vi "FunctionGeneratorMatrix_Add_Value.vi"(9 "Y Value":T1, 10 "X Value":dbl, 11 "in FUNC_GEN_MATRIX":T2) -> (0 "Error":bool, 3 "out FUNC_GEN_MATRIX":T2)   [LabVIEW 2019, in "Trajectory_Library.lvlib"]
doc: "Insert new X, Y pair into an existing Function Generator Matrix data cluster.\n\nInputs:\n - Input Funct Gen Matrix -- Data cluster\n - X Value -- New X value\n - Y Value -- New Y matrix\n\nOutputs:\n - Function Generator Matrix -- Updated data cluster\n - Error -- Set true if an error occured. This is set when the size of the Y matrix does not match the definiton of this function generator."
uses:
  Trajectory_Library.lvlib
  TypeDef/FUNCTION_GENERATOR_MATRIX.ctl
  <vilib>/Analysis/Matrix/Datatypes/RealMatrix.ctl
  <vilib>/gmath/NI_Gmath.lvlib
  <vilib>/Analysis/Matrix/NI_Matrix.lvlib
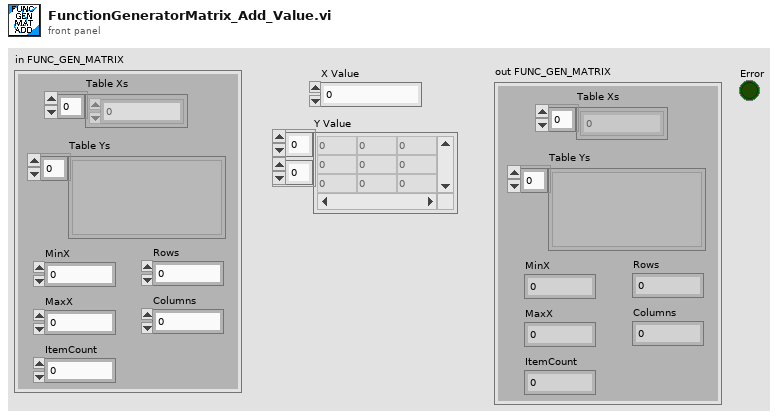
[diagram p1: front panel]
types:
  T1 = typedef "NI_Matrix.lvlib/RealMatrix.ctl" = dbl[][]
  T2 = typedef "Trajectory_Library.lvlib/FUNCTION_GENERATOR_MATRIX.ctl" = cluster{"Table Xs":dbl[], "Table Ys":variant[], "MinX":dbl, "MaxX":dbl, "ItemCount":i32, "Rows":i32, "Columns":i32}
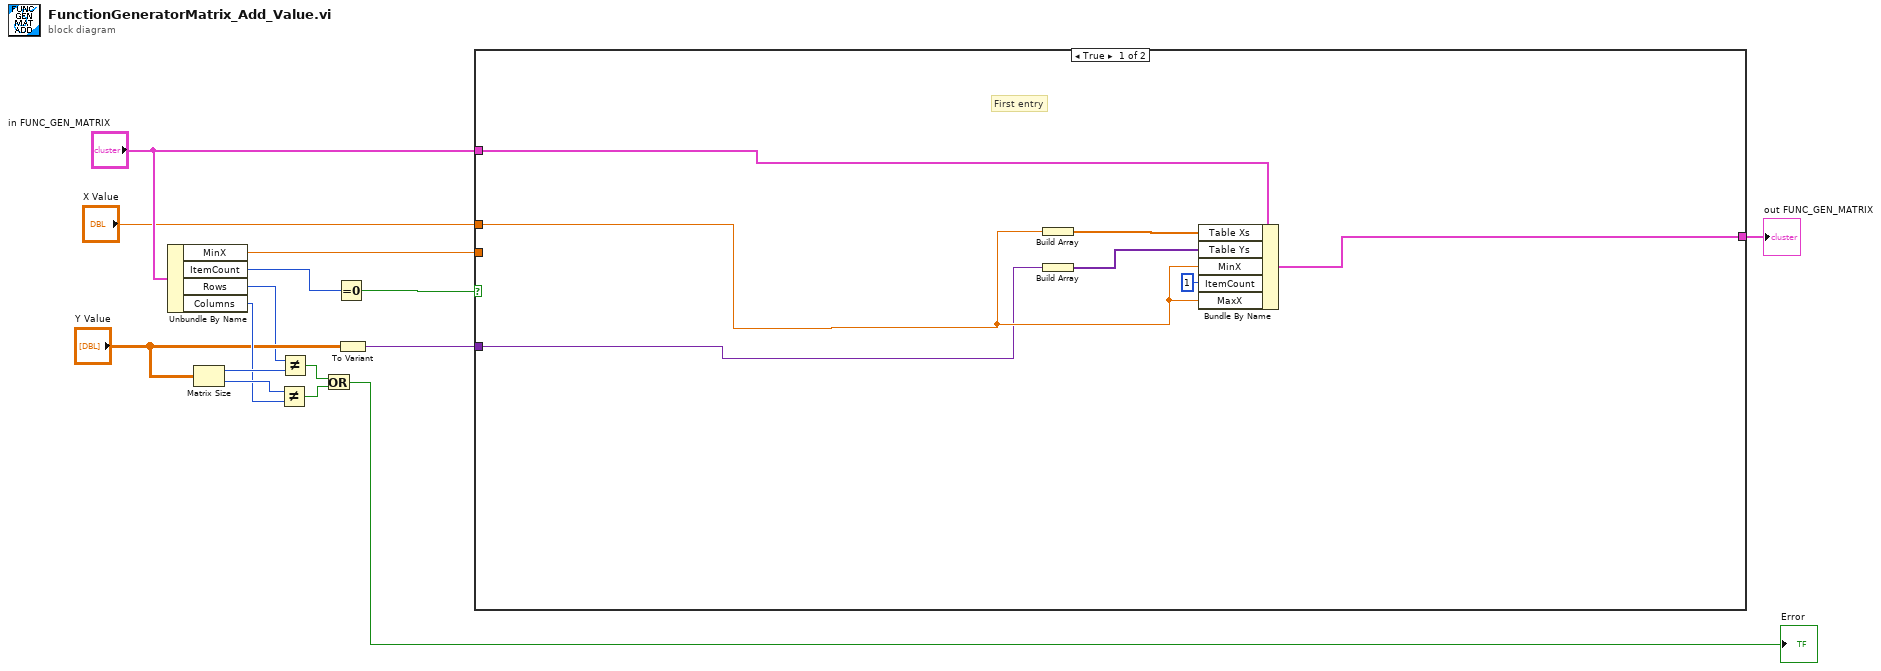
[diagram p0: block diagram]
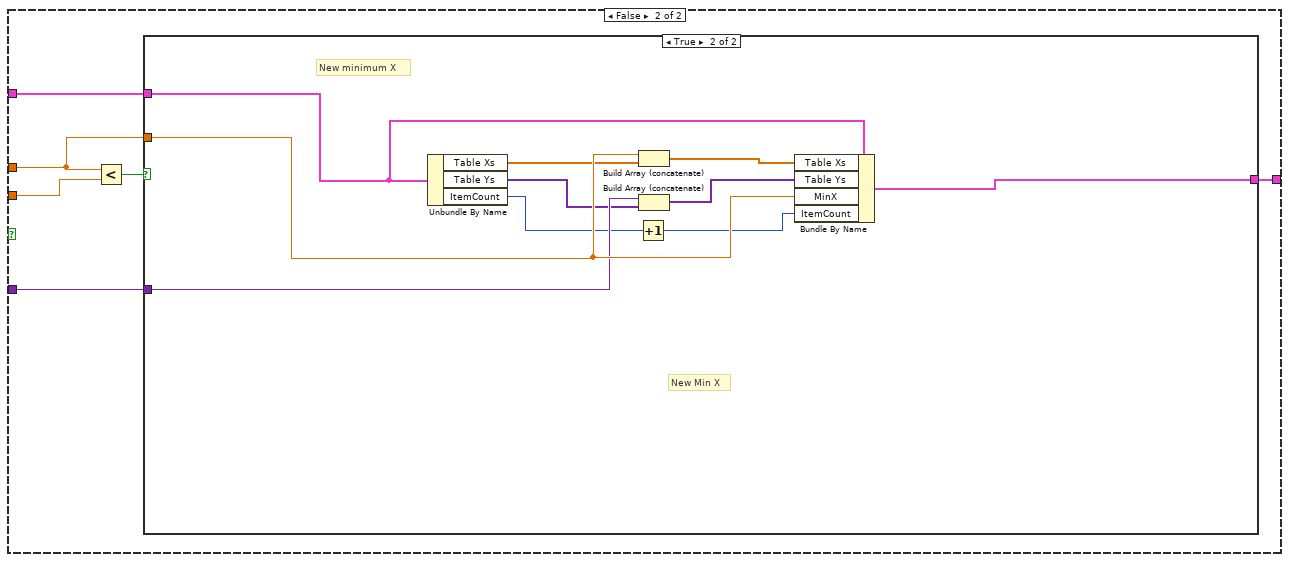
[diagram p2: hidden frame]
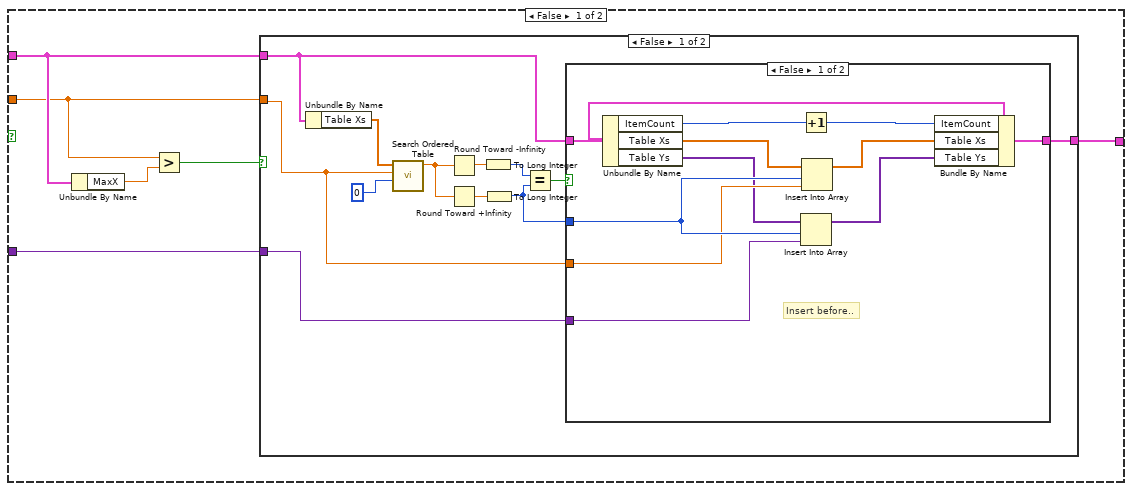
[diagram p3: hidden frame]
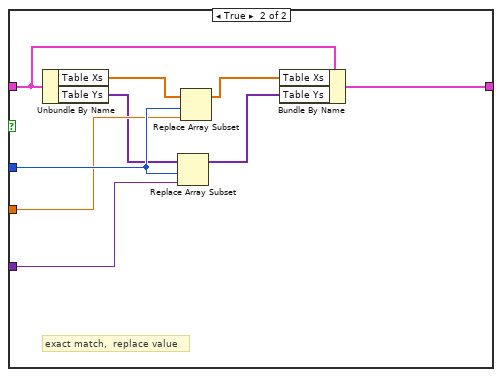
[diagram p4: hidden frame]
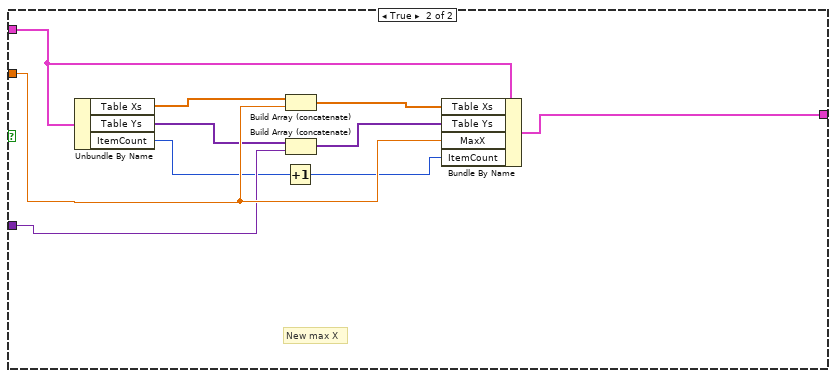
[diagram p5: hidden frame]
diagram:
  n1 = Unbundle By Name("in FUNC_GEN_MATRIX") -> ("MinX"=w15:dbl, "ItemCount"=w2:i32, "Rows"=w3:i32, "Columns"=w9:i32)
  n2 = Matrix Size(0:"Y Value") -> (1:w11:i32, 2:w10:i32)
  n3 = Not Equal?(x=w10, y=w9) -> (x != y?=w7:bool)
  n4 = Not Equal?(x=w3, y=w11) -> (x != y?=w8:bool)
  n5 = Or(x=w8, y=w7) -> (x .or. y?=→"Error":bool)
  n6 = Equal To 0?(x=w2) -> (x = 0?=w1:bool)
  n7 = To Variant(anything="Y Value") -> (Variant=w4:variant)
  n8 = case shown="True" w1 {
    tunnel: w15 -> [_ w28]
    tunnel: "in FUNC_GEN_MATRIX" -> [w22 w26]
    tunnel: "X Value" -> [w21 w25]
    tunnel: [w19 w24] -> w12
    tunnel: w4 -> [w20 w23]
    frame True {
      # "First entry"
      n9 = Build Array(w21) -> (w18:dbl[])
      n10 = Build Array(w20) -> (w17:variant[])
      n11 = Bundle By Name(cluster=w22, "Table Xs"=w18, "Table Ys"=w17, "MinX"=w21, "ItemCount"=1, "MaxX"=w21) -> (w19:T2)
    }
    frame False {
      n12 = Less?(x=w25, y=w28) -> (x < y?=w27:bool)
      n13 = case shown="True" w27 {
        tunnel: w26 -> [w33 w86]
        tunnel: w25 -> [w31 w85]
        tunnel: w23 -> [w30 w84]
        tunnel: [w32 w83] -> w24
        frame False {
          n14 = Unbundle By Name(w33) -> ("MaxX"=w34:dbl)
          n15 = Greater?(x=w31, y=w34) -> (0:w29:bool)
          n16 = case shown="False" w29 {
            tunnel: w33 -> [w39 w76]
            tunnel: [w35 w75] -> w32
            tunnel: w31 -> [w37 w74]
            tunnel: w30 -> [w36 w73]
            frame False {
              n17 = Unbundle By Name(w39) -> ("Table Xs"=w45:dbl[])
              n18 = call <vilib>:"Search Ordered Table.vi"("starting index"=0, "x value"=w37, "ordered x array"=w45) -> ("fractional index"=w44:dbl)  [unwired: 8 in]
              n19 = Round Toward -Infinity(1:w44) -> (0:w42:dbl)
              n20 = Round Toward +Infinity(x=w44) -> (ceil(x): smallest int >= x=w43:dbl)
              n21 = To Long Integer(number=w42) -> (32bit integer=w41:i32)
              n22 = To Long Integer(number=w43) -> (32bit integer=w38:i32)
              n23 = Equal?(x=w41, y=w38) -> (x = y?=w40:bool)
              n24 = case shown="False" w40 {
                tunnel: w39 -> [w54 w66]
                tunnel: w38 -> [w57 w65]
                tunnel: w37 -> [w56 w64]
                tunnel: w36 -> [w55 w63]
                tunnel: [w53 w62] -> w35
                frame False {
                  # "Insert before.."
                  n25 = Unbundle By Name(w54) -> ("ItemCount"=w52:i32, "Table Xs"=w50:dbl[], "Table Ys"=w49:variant[])
                  n26 = Increment(x=w52) -> (x+1=w51:i32)
                  n27 = Insert Into Array(array=w49, index=w57, new element=w55) -> (w47:variant[])
                  n28 = Insert Into Array(array=w50, index=w57, new element=w56) -> (w48:dbl[])
                  n29 = Bundle By Name(cluster=w54, "ItemCount"=w51, "Table Xs"=w48, "Table Ys"=w47) -> (w53:T2)
                }
                frame True {
                  # "exact match,  replace value"
                  n30 = Unbundle By Name(w66) -> ("Table Xs"=w61:dbl[], "Table Ys"=w60:variant[])
                  n31 = Replace Array Subset(array=w60, new element=w63, index=w65) -> (w58:variant[])
                  n32 = Replace Array Subset(array=w61, new element=w64, index=w65) -> (w59:dbl[])
                  n33 = Bundle By Name(cluster=w66, "Table Xs"=w59, "Table Ys"=w58) -> (w62:T2)
                }
              }
            }
            frame True {
              # "New max X"
              n34 = Unbundle By Name(w76) -> ("Table Xs"=w68:dbl[], "Table Ys"=w67:variant[], "ItemCount"=w70:i32)
              n35 = Increment(x=w70) -> (x+1=w69:i32)
              n36 = Build Array (concatenate)(w68, w74) -> (w72:dbl[])
              n37 = Build Array (concatenate)(w67, w73) -> (w71:variant[])
              n38 = Bundle By Name(cluster=w76, "Table Xs"=w72, "Table Ys"=w71, "MaxX"=w74, "ItemCount"=w69) -> (w75:T2)
            }
          }
        }
        frame True {
          # "New Min X"
          # "New minimum X"
          n39 = Unbundle By Name(w86) -> ("Table Xs"=w82:dbl[], "Table Ys"=w79:variant[], "ItemCount"=w78:i32)
          n40 = Increment(x=w78) -> (x+1=w77:i32)
          n41 = Build Array (concatenate)(w85, w82) -> (w81:dbl[])
          n42 = Build Array (concatenate)(w84, w79) -> (w80:variant[])
          n43 = Bundle By Name(cluster=w86, "Table Xs"=w81, "Table Ys"=w80, "MinX"=w85, "ItemCount"=w77) -> (w83:T2)
        }
      }
    }
  }
  "out FUNC_GEN_MATRIX" <- w12
